vi "Test_Commands.vi"(11 "Initial Command":T1[](array[typedef])=[enum."Shutdown", enum."Switch On", enum."Disable Voltage", enum."Quick Stop", enum."Disable Op", enum."Enable Op", enum."Fault Reset"]) -> (1 "Pass?":bool[](array[boolean]), 2 "ControlWord":u16[](array[numeric]) format="%08b", 3 "WordToCommand":T1[](array[typedef]))   [LabVIEW 2017, in "WordManipulationTests.lvlib"]
uses:
  WordManipulationTests.lvlib
  Utilities/Controlword_Commands.ctl
  Utilities/WordManipulationLibrary.lvlib
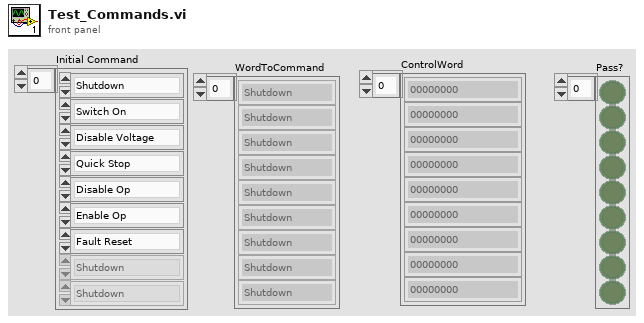
[diagram p1: front panel]
types:
  T1 = typedef "WordManipulationLibrary.lvlib/Controlword_Commands.ctl" = enum16{"Shutdown", "Switch On", "Disable Voltage", "Quick Stop", "Disable Op", "Enable Op", "Fault Reset", "Error"}
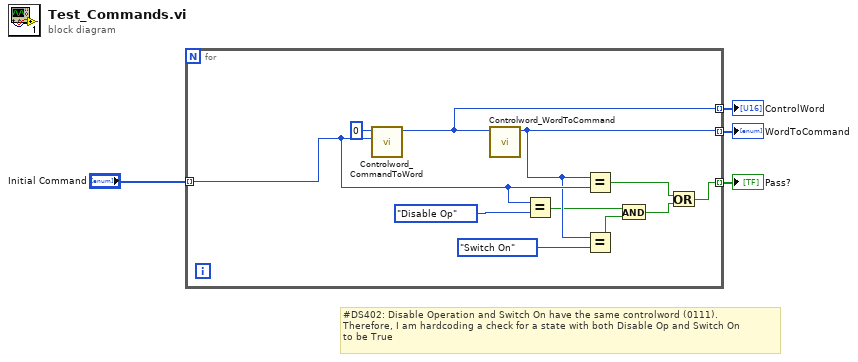
[diagram p0: block diagram]
diagram:
  # "#DS402: Disable Operation and Switch On have the same controlword (0111). \nTherefore, I am hardcoding a check for a state with both Disable Op and Switch On\nto be True"
  n1 = for {
    tunnel: [w5] -> w4 mode=indexing
    tunnel: [w10] -> w3 mode=indexing
    tunnel: [w14] -> w2 mode=indexing
    tunnel: "Initial Command" -> [w13] mode=indexing
    n2 = call "Controlword_CommandToWord.vi"("Device Control Command"=w13, "ControlWord In"=u16 0) -> ("ControlWord Out"=w14:u16)  [unwired: 9 in]
    n3 = call "Controlword_WordToCommand.vi"("Controlword"=w14) -> ("Device Control Command"=w10:T1)  [unwired: 10 in]
    n4 = Equal?(x=w13, y=Controlword_Commands."Disable Op") -> (x = y?=w9:bool)
    n5 = Equal?(x=w10, y=w13) -> (x = y?=w6:bool)
    n6 = Equal?(x=w10, y=Controlword_Commands."Switch On") -> (x = y?=w8:bool)
    n7 = And(x=w9, y=w8) -> (x .and. y?=w7:bool)
    n8 = Or(x=w6, y=w7) -> (x .or. y?=w5:bool)
  }
  "Pass?" <- w4
  "WordToCommand" <- w3
  "ControlWord" <- w2
